vi "Generate Scale List Menu.vi"(9 "Scale List Select Index":i32, 10 "Item Names":string[](array[string]), 11 "Menu in":refnum<k9>) -> ()   [LabVIEW 2020, in "Data Viewer.lvlib"]
uses:
  Data Viewer.lvlib
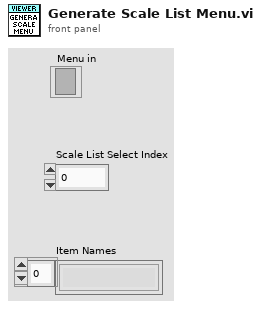
[diagram p1: front panel]
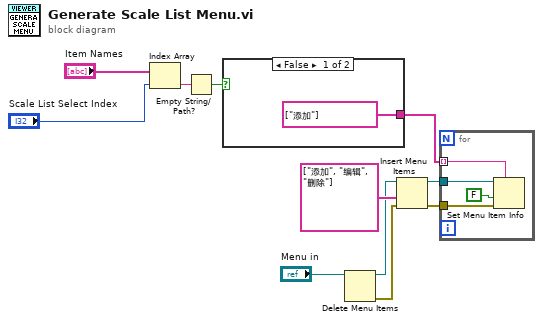
[diagram p0: block diagram]
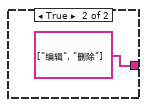
[diagram p2: hidden frame]
diagram:
  n1 = Index Array(array="Item Names", index="Scale List Select Index") -> (element=w8:string)
  n2 = Empty String/Path?(string/path=w8) -> (empty?=w9:bool)
  n3 = case shown="False" w9 {
    tunnel: [string[] ["添加"] ("item names") string[] ["编辑", "删除"] ("item names")] -> w1
    frame False {
    }
    frame True {
    }
  }
  n4 = Delete Menu Items(9:"Menu in") -> (0:w10:errorcluster, 3:w5:refnum<k9>)  [unwired: 3 in]
  n5 = Insert Menu Items(6:w10, 7:string[] ["添加", "编辑", "删除"] ("item names"), 9:w5) -> (0:w2:errorcluster, 3:w3:refnum<k9>)  [unwired: 3 in, 1 out]
  n6 = for {
    tunnel: w3 -> [w17]
    tunnel: w2 -> [w16]
    tunnel: w1 -> [w14] mode=indexing
    n7 = Set Menu Item Info(7:w14, 8:w16, 9:FALSE ("enabled"), 11:w17) -> ()  [unwired: 3 in, 2 out]
  }
